vi "XBOX_Joystick_Name.vi"(9 "POVs":i16[](array[numeric]), 10 "Buttons":bool[](array[boolean]), 11 "Axes":dbl[](array[numeric])) -> (2 "Named Axes":T1, 3 "Named Buttons":T2)   [LabVIEW 2019, in "ArgosLib.lvlib"]
uses:
  ArgosLib.lvlib
  TypeDefs/XBoxButtons_Type.ctl
  TypeDefs/XBoxAxes_Type.ctl
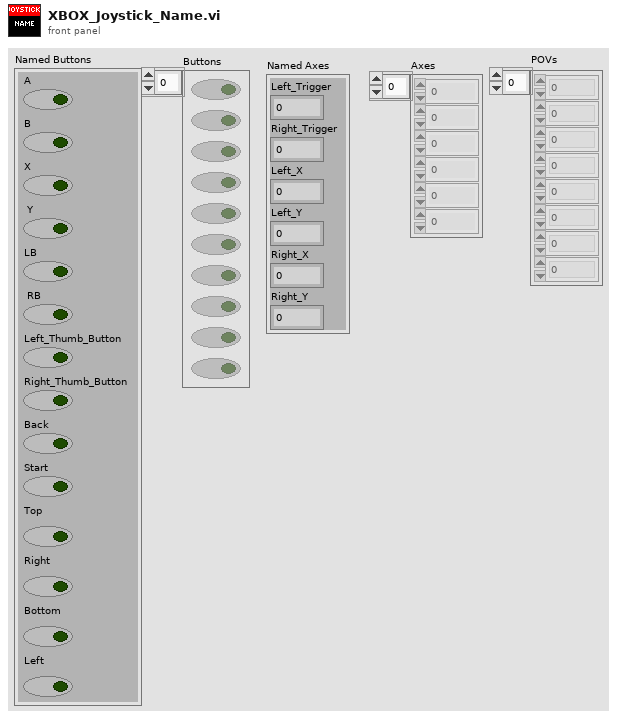
[diagram p1: front panel]
types:
  T1 = typedef "ArgosLib.lvlib/XBoxAxes_Type.ctl" = cluster{"Left_Trigger":dbl, "Right_Trigger ":dbl, "Left_X":dbl, "Left_Y":dbl, "Right_X":dbl, "Right_Y":dbl}
  T2 = typedef "ArgosLib.lvlib/XBoxButtons_Type.ctl" = cluster{"A":bool, "B":bool, "X":bool, " Y":bool, "LB":bool, " RB":bool, "Left_Thumb_Button":bool, "Right_Thumb_Button":bool, "Back":bool, "Start":bool, "Top":bool, "Right":bool, "Bottom":bool, "Left":bool}
  T3 = cluster{"Axes[0]":dbl, "Axes[1]":dbl, "Axes[2]":dbl, "Axes[3]":dbl, "Axes[4]":dbl, "Axes[5]":dbl}
  T4 = cluster{"Buttons[0]":bool, "Buttons[1]":bool, "Buttons[2]":bool, "Buttons[3]":bool, "Buttons[4]":bool, "Buttons[5]":bool, "Buttons[6]":bool, "Buttons[7]":bool, "Buttons[8]":bool, "Buttons[9]":bool}
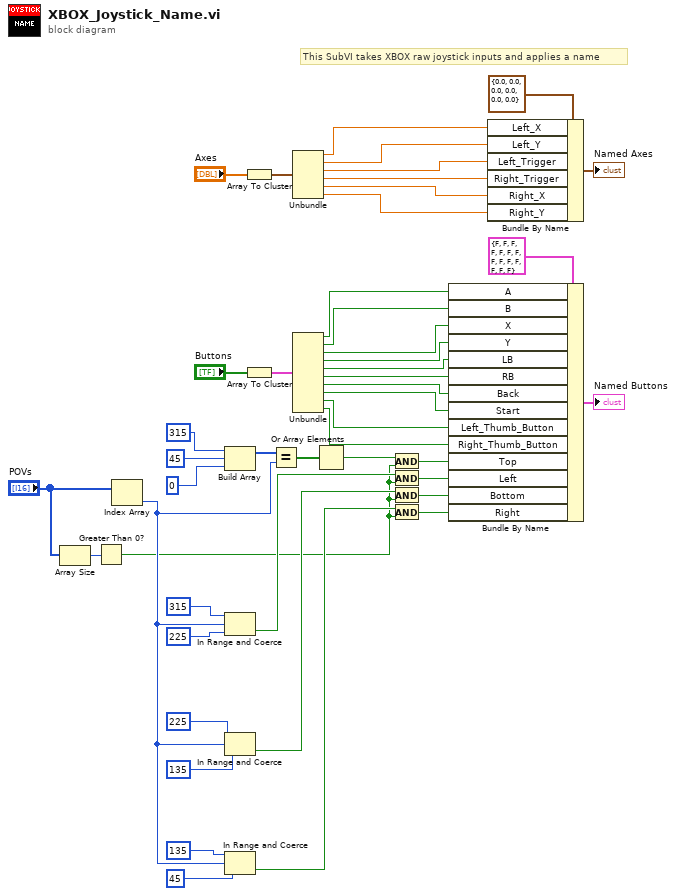
[diagram p0: block diagram]
diagram:
  # "This SubVI takes XBOX raw joystick inputs and applies a name"
  n1 = Array Size(array="POVs") -> (size(s)=w9:i32)
  n2 = Greater Than 0?(x=w9) -> (x > 0?=w3:bool)
  n3 = Index Array(array="POVs") -> (element=w12:i16)  [unwired: 1 in]
  n4 = Build Array(i16 315 ("upper limit"), i16 45 ("element"), i16 0 ("element")) -> (w13:i16[])
  n5 = In Range and Coerce(upper limit=i16 315, x=w12, lower limit=i16 225) -> (In Range?=w19:bool)  [unwired: 1 out]
  n6 = In Range and Coerce(upper limit=i16 225, x=w12, lower limit=i16 135) -> (In Range?=w18:bool)  [unwired: 1 out]
  n7 = In Range and Coerce(upper limit=i16 135, x=w12, lower limit=i16 45) -> (In Range?=w4:bool)  [unwired: 1 out]
  n8 = Array To Cluster(array="Axes") -> (cluster=w32:T3)
  n9 = Array To Cluster(array="Buttons") -> (cluster=w29:T4)
  n10 = Equal?(x=w13, y=w12) -> (x = y?=w14:bool[])
  n11 = Unbundle(w32) -> ("Axes[0]"=w44:dbl, "Axes[1]"=w2:dbl, "Axes[2]"=w45:dbl, "Axes[3]"=w46:dbl, "Axes[4]"=w47:dbl, "Axes[5]"=w1:dbl)
  n12 = Unbundle(w29) -> ("Buttons[0]"=w34:bool, "Buttons[1]"=w35:bool, "Buttons[2]"=w36:bool, "Buttons[3]"=w37:bool, "Buttons[4]"=w38:bool, "Buttons[5]"=w39:bool, "Buttons[6]"=w40:bool, "Buttons[7]"=w41:bool, "Buttons[8]"=w42:bool, "Buttons[9]"=w28:bool)
  n13 = Or Array Elements(Boolean array=w14) -> (logical OR=w11:bool)
  n14 = And(x=w11, y=w3) -> (x .and. y?=w8:bool)
  n15 = And(x=w19, y=w3) -> (x .and. y?=w7:bool)
  n16 = And(x=w18, y=w3) -> (x .and. y?=w6:bool)
  n17 = And(x=w4, y=w3) -> (x .and. y?=w5:bool)
  n18 = Bundle By Name(cluster=T2 {"A"=FALSE, "B"=FALSE, "X"=FALSE, " Y"=FALSE, "LB"=FALSE, " RB"=FALSE, "Left_Thumb_Button"=FALSE, "Right_Thumb_Button"=FALSE, "Back"=FALSE, "Start"=FALSE, "Top"=FALSE, "Right"=FALSE, "Bottom"=FALSE, "Left"=FALSE}, "A"=w34, "B"=w35, "X"=w36, "Y"=w37, "LB"=w38, "RB"=w39, "Back"=w40, "Start"=w41, "Left_Thumb_Button"=w42, "Right_Thumb_Button"=w28, "Top"=w8, "Left"=w7, "Bottom"=w6, "Right"=w5) -> (→"Named Buttons":T2)
  n19 = Bundle By Name(cluster=T1 {"Left_Trigger"=0.0, "Right_Trigger "=0.0, "Left_X"=0.0, "Left_Y"=0.0, "Right_X"=0.0, "Right_Y"=0.0}, "Left_X"=w44, "Left_Y"=w2, "Left_Trigger"=w45, "Right_Trigger"=w46, "Right_X"=w47, "Right_Y"=w1) -> (→"Named Axes":T1)
